vi "UE_Target_Error.vi"(1 "actual":dbl, 2 "target":dbl) -> (0 "error":dbl)   [LabVIEW 2026]
doc: "INTENT: Compute signed target minus feedback error. INPUTS: target (double), actual (double). OUTPUTS: error (double). DESIGN CONSTRAINT: REQUIREMENTS: SRS-F-005. No physical hardware side effects. Acceptance requires native LabVIEW compilation and behavioral testing."
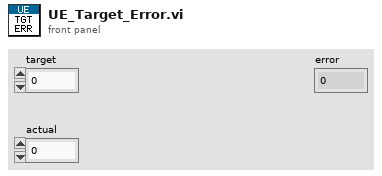
[diagram p1: front panel]
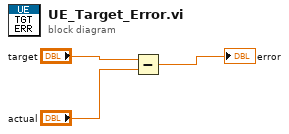
[diagram p0: block diagram]
diagram:
  n1 = Subtract(x="target", y="actual") -> (x-y=→"error":dbl)
